vi "Write events.vi"(8 "error in (no error)":errorcluster, 10 "ZM-HWM-EVENTS":T1, 11 "ZM-HWM-hardware_manager in":refnum<class "ZM-HWM-hardware_manager.lvclass">) -> (0 "error out":errorcluster, 3 "ZM-HWM-hardware_manager out":refnum<class "ZM-HWM-hardware_manager.lvclass">)   [LabVIEW 2020, in "ZM-HWM-hardware_manager.lvlib" / "ZM-HWM-hardware_manager.lvclass"]
doc: "Writes one field of this class's private data. Generated by lvai_create_accessors from the class private data control."
uses:
  ZM-HWM-hardware_manager.lvclass
  ZM-HWM-hardware_manager.lvclass/ZM-HWM-hardware_manager.ctl
  ZM-HWM-EVENTS.ctl
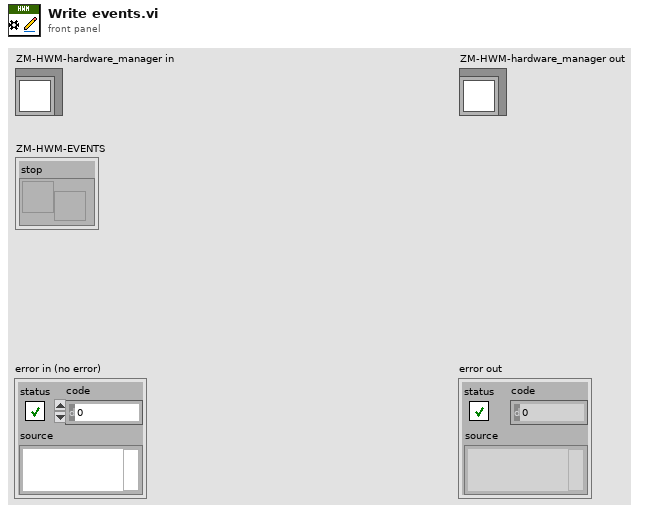
[diagram p1: front panel]
types:
  T1 = typedef "ZM-HWM-hardware_manager.lvlib/ZM-HWM-hardware_manager.lvclass/ZM-HWM-EVENTS.ctl" = cluster{"stop":refnum<user-event>}
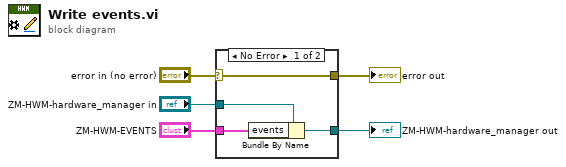
[diagram p0: block diagram]
diagram:
  n1 = case shown="No Error" "error in (no error)" {
    selector: "error in (no error)" -> [w9 w10]
    tunnel: [w9 w10] -> w4
    tunnel: [w7 w11] -> w2
    tunnel: "ZM-HWM-hardware_manager in" -> [w8 w11]
    tunnel: "ZM-HWM-EVENTS" -> [w6 _]
    frame No Error {
      n2 = Bundle By Name(cluster=w8, "events"=w6) -> (w7:refnum<class "ZM-HWM-hardware_manager.lvclass">)
    }
    frame Error {
    }
  }
  "error out" <- w4
  "ZM-HWM-hardware_manager out" <- w2
